vi "xnet_canopen_request_tpdo.vi"(8 "error in (no error)":errorcluster, 10 "tpdo_number":u16, 11 "xnet_co_handle_in":u64) -> (0 "error out":errorcluster, 3 "xnet_co_handle":u64)   [LabVIEW 2023, in "xnet_canopen.lvlib"]
uses:
  <vilib>/Utility/error.llb/Error Cluster From Error Code.vi
  xnet_canopen.lvlib
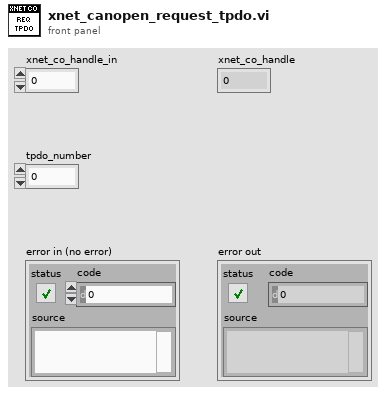
[diagram p1: front panel]
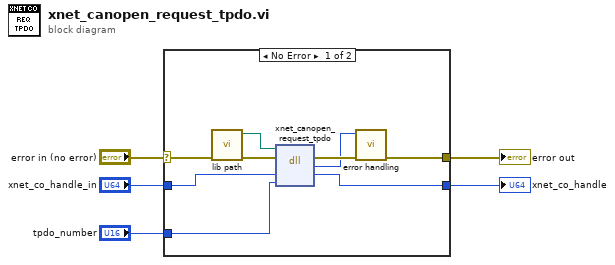
[diagram p0: block diagram]
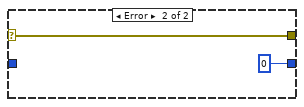
[diagram p2: hidden frame]
diagram:
  n1 = case shown="No Error" "error in (no error)" {
    selector: "error in (no error)" -> [w12 w15]
    tunnel: [w10 w15] -> w4
    tunnel: [w8 u64 0 ("phandle")] -> w3
    tunnel: "xnet_co_handle_in" -> [w7 _]
    tunnel: "tpdo_number" -> [w6 _]
    frame No Error {
      n2 = call "lib path.vi"() -> ("lib path"=w13:path)  [unwired: 11 in]
      n3 = dll-call lib="?" fn="xnet_canopen_request_tpdo"(path in=w13, error in=w12, "handle"=w7, "tpdo_number"=w6) -> (error out=w11:errorcluster, "return type"=w9:i32, "handle"=w8:u64)  [unwired: 2 in, 1 out]
      n4 = call "error handling.vi"("error in (no error)"=w11, "return val"=w9) -> ("error out"=w10:errorcluster)  [unwired: 9 in]
    }
    frame Error {
    }
  }
  "error out" <- w4
  "xnet_co_handle" <- w3
